vi "RFH-utility-average_common_format.vi"(10 "common array in":T1[](array[typedef])) -> (2 "Common Format":T1)   [LabVIEW 2020, in "RFH-Reflection_File_Handler.lvlib"]
doc: "Averages an array of Common Format clusters into one."
uses:
  RFH-Reflection_File_Handler.lvlib
  RFH-common_data_format.ctl
panel:
  out "Waveform Graph 2":dbl[](graph)
  out "Waveform Graph":dbl[][](graph)
  out "x = y?":bool
  out "Samples":i32
  out "Array 4":dbl[](array[numeric])
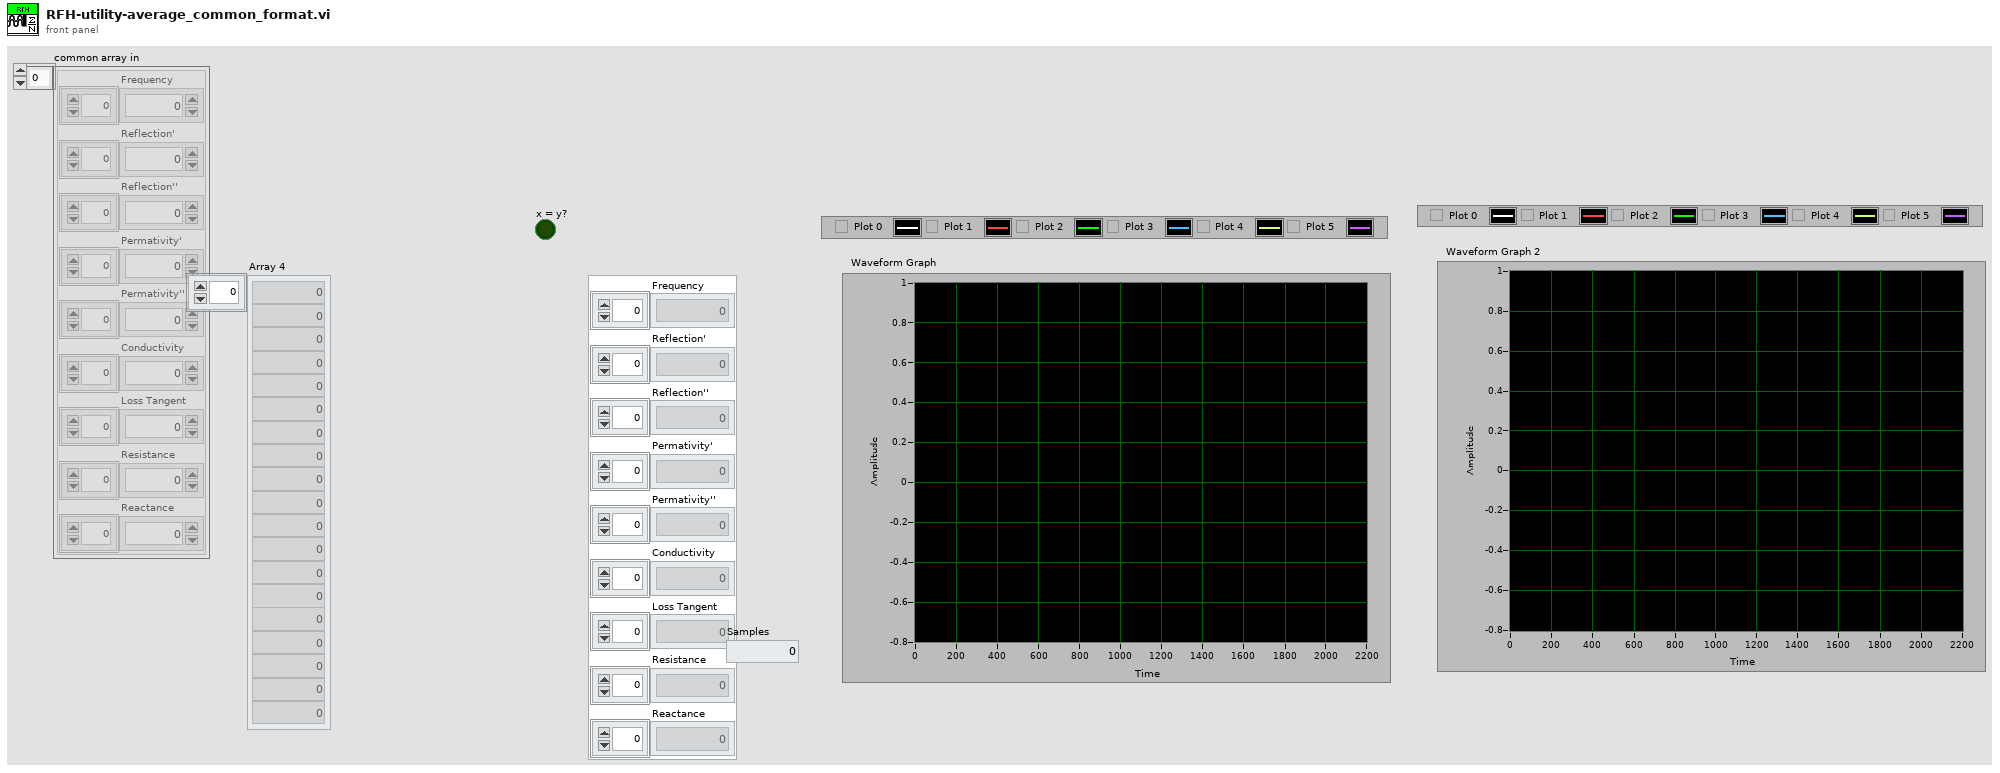
[diagram p1: front panel]
types:
  T1 = typedef "RFH-Reflection_File_Handler.lvlib/RFH-common_data_format.ctl" = cluster{"Frequency":dbl[], "Reflection'":dbl[], "Reflection''":dbl[], "Permativity'":dbl[], "Permativity''":dbl[], "Conductivity":dbl[], "Loss Tangent":dbl[], "Resistance":dbl[], "Reactance":dbl[]}
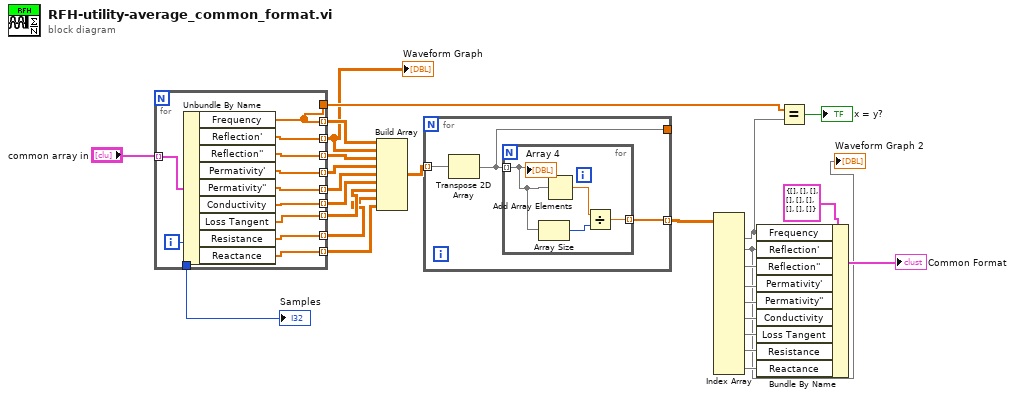
[diagram p0: block diagram]
diagram:
  n1 = for {
    tunnel: "common array in" -> [w37] mode=indexing
    tunnel: [w31] -> w3 mode=indexing
    tunnel: [w36] -> w2 mode=indexing
    tunnel: [w35] -> w26 mode=indexing
    tunnel: [w34] -> w25 mode=indexing
    tunnel: [w33] -> w24 mode=indexing
    tunnel: [w32] -> w22
    tunnel: [w31] -> w13
    tunnel: [w30] -> w7 mode=indexing
    tunnel: [w29] -> w6 mode=indexing
    tunnel: [w28] -> w5 mode=indexing
    tunnel: [w27] -> w4 mode=indexing
    i -> [w32]
    n2 = Unbundle By Name(w37) -> ("Frequency"=w31:dbl[], "Reflection'"=w36:dbl[], "Reflection''"=w35:dbl[], "Permativity'"=w34:dbl[], "Permativity''"=w33:dbl[], "Conductivity"=w30:dbl[], "Loss Tangent"=w29:dbl[], "Resistance"=w28:dbl[], "Reactance"=w27:dbl[])
  }
  "Samples" <- w22
  "Waveform Graph" <- w2
  n3 = Build Array(w3, w2, w26, w25, w24, w7, w6, w5, w4) -> (w23:dbl[][][])
  n4 = for {
    tunnel: w23 -> [w39] mode=indexing
    tunnel: [w40] -> w20 mode=indexing
    tunnel: [w38] -> _
    n5 = Transpose 2D Array(2D array=w39) -> (transposed array=w38:dbl[][])
    n6 = for {
      tunnel: w38 -> [w42] mode=indexing
      tunnel: [w41] -> w40 mode=indexing
      n7 = Array Size(array=w42) -> (size(s)=w44:i32)
      n8 = Add Array Elements(numeric array=w42) -> (sum=w43:dbl)
      n9 = Divide(x=w43, y=w44) -> (x/y=w41:dbl)
      "Array 4" <- w42
    }
  }
  n10 = Index Array(array=w20) -> (element #1=w14:dbl[], element #2=w1:dbl[], element #3=w17:dbl[], element #4=w16:dbl[], element #5=w15:dbl[], element #6=w8:dbl[], element #7=w9:dbl[], element #8=w10:dbl[], element #9=w11:dbl[])  [unwired: 18 in]
  "Waveform Graph 2" <- w1
  n11 = Bundle By Name(cluster=T1 {"Frequency"=[], "Reflection'"=[], "Reflection''"=[], "Permativity'"=[], "Permativity''"=[], "Conductivity"=[], "Loss Tangent"=[], "Resistance"=[], "Reactance"=[]} ("Common Format"), "Frequency"=w14, "Reflection'"=w1, "Reflection''"=w17, "Permativity'"=w16, "Permativity''"=w15, "Conductivity"=w8, "Loss Tangent"=w9, "Resistance"=w10, "Reactance"=w11) -> (→"Common Format":T1)
  n12 = Equal?(x=w13, y=w14) -> (x = y?=→"x = y?":bool)
